vi "VIH HelpGen - FILE - Build Absolute Path.vi"(7 "Root Path":path, 10 "Allow Empty Path (T)":bool=TRUE, 11 "Path in":path) -> (3 "Path out":path)   [LabVIEW 2014]
doc: "::: VI Helpeks :::\nCopyright (c) 2000-2026 Konstantin Shifershteyn. All rights reserved."
panel:
  # "VI Helpeks\nCopyright (c) 2012-2026 Konstantin Shifershteyn"
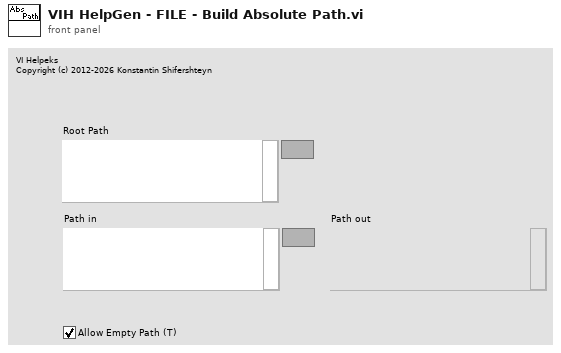
[diagram p1: front panel]
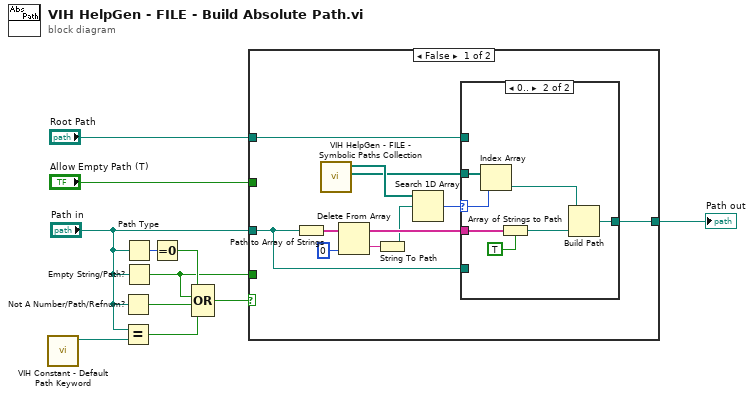
[diagram p0: block diagram]
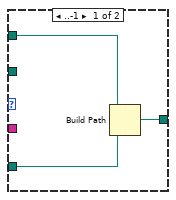
[diagram p2: hidden frame]
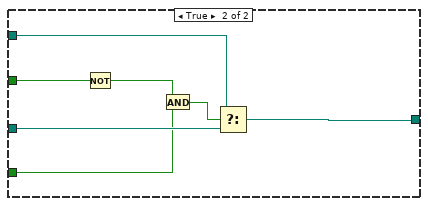
[diagram p3: hidden frame]
diagram:
  n1 = call "VIH Constant - Default Path Keyword.vi"() -> ("<default> path"=w1:path)  [unwired: 11 in]
  n2 = Not A Number/Path/Refnum?(number/path/refnum="Path in") -> (NaN/Path/Refnum?=w6:bool)
  n3 = Equal?(x="Path in", y=w1) -> (x = y?=w7:bool)
  n4 = Path Type(1:"Path in") -> (0:w8:i16)
  n5 = Empty String/Path?(string/path="Path in") -> (empty?=w3:bool)
  n6 = Equal To 0?(x=w8) -> (x = 0?=w5:bool)
  n7 = Compound Arithmetic op=OR(w5, w3, w6, w7) -> (w4:bool)
  n8 = case shown="False" w4 {
    tunnel: "Path in" -> [w13 w38]
    tunnel: [w15 w39] -> w11
    tunnel: "Root Path" -> [w12 w37]
    tunnel: w3 -> [_ w36]
    tunnel: "Allow Empty Path (T)" -> [_ w35]
    frame False {
      n9 = Path to Array of Strings(0:w13) -> (2:w22:string[])  [unwired: 1 out]
      n10 = call "VIH HelpGen - FILE - Symbolic Paths Collection.vi"() -> ("Absolute Paths"=w17:path[], "Symbolic Paths"=w18:path[])  [unwired: 10 in]
      n11 = Delete From Array(array=w22, index=0) -> (deleted portion=w19:string, array with subset deleted=w20:string[])  [unwired: 1 in]
      n12 = String To Path(string=w19) -> (path=w16:path)
      n13 = Search 1D Array(1D array=w18, element=w16) -> (index of element=w14:i32)  [unwired: 1 in]
      n14 = case shown="0.." w14 {
        selector: w14 -> [_ w26]
        tunnel: w20 -> [_ w32]
        tunnel: w17 -> [_ w30]
        tunnel: [w25 w28] -> w15
        tunnel: w13 -> [w24 _]
        tunnel: w12 -> [w23 _]
        frame ..-1 {
          n15 = Build Path(base path=w23, name or relative path=w24) -> (appended path=w25:path)
        }
        frame 0.. {
          n16 = Index Array(array=w30, index=w26) -> (element=w27:path)
          n17 = Array of Strings to Path(0:w32, 1:TRUE) -> (2:w29:path)
          n18 = Build Path(base path=w27, name or relative path=w29) -> (appended path=w28:path)
        }
      }
    }
    frame True {
      n19 = Not(x=w35) -> (.not. x?=w34:bool)
      n20 = And(x=w34, y=w36) -> (x .and. y?=w33:bool)
      n21 = Select(t=w37, s=w33, f=w38) -> (s? t:f=w39:path)
    }
  }
  "Path out" <- w11
